vi "Call Check and Download Bitfile.vi"(8 "error in":errorcluster, 9 "Target IP Address":string, 10 "Bitfile Path":path, 11 "Slave Ref":string) -> (0 "error out":errorcluster)   [LabVIEW 2020, in "SEECD System Explorer.lvlib"]
uses:
  SEECD System Explorer.lvlib
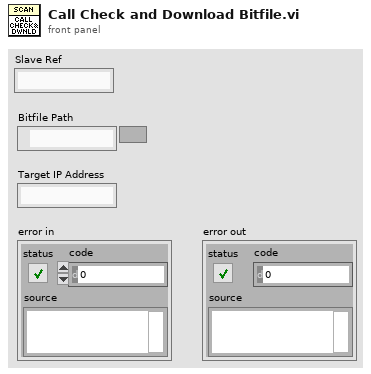
[diagram p1: front panel]
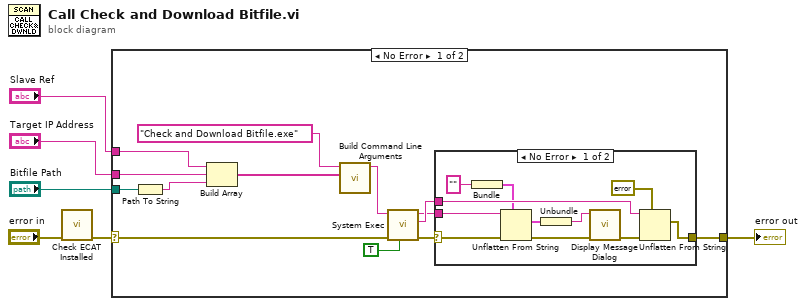
[diagram p0: block diagram]
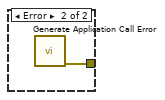
[diagram p2: hidden frame]
diagram:
  n1 = call "Check ECAT Installed.vi"("error in (no error)"="error in") -> ("error out"=w1:errorcluster)  [unwired: 10 in]
  n2 = case shown="No Error" w1 {
    selector: w1 -> [w19 w32]
    tunnel: [w9 w32] -> w2
    tunnel: "Slave Ref" -> [w16 _]
    tunnel: "Target IP Address" -> [w15 _]
    tunnel: "Bitfile Path" -> [w17 _]
    frame No Error {
      n3 = Path To String(path=w17) -> (string=w14:string)
      n4 = Build Array(w16, w15, w14) -> (w13:string[])
      n5 = call "Build Command Line Arguments.vi"("Arguments"=w13, "Executable File Name"="Check and Download Bitfile.exe" ("name or relative path")) -> ("Command Line"=w11:string)  [unwired: 9 in]
      n6 = call <vilib>:"System Exec.vi"("run minimized? (F)"=TRUE, "error in (no error)"=w19, "command line"=w11) -> ("error out"=w10:errorcluster, "standard error"=w8:string, "standard output"=w7:string)  [unwired: 5 in, 1 out]
      n7 = case shown="No Error" w10 {
        selector: w10 -> [w26 _]
        tunnel: [w29 w31] -> w9
        tunnel: w8 -> [w28 _]
        tunnel: w7 -> [w23 _]
        frame No Error {
          n8 = Bundle("") -> (w24:cluster{string})  [unwired: 1 in]
          n9 = Unflatten From String(type=w24, binary string=w23, error in (no error)=w26) -> (value=w21:cluster{string}, error out=w25:errorcluster)  [unwired: 2 in, 1 out]
          n10 = Unbundle(w21) -> (w20:string)
          n11 = call "Display Message Dialog.vi"("error in"=w25, "Message to display"=w20) -> ("error out"=w27:errorcluster)  [unwired: 9 in]
          n12 = Unflatten From String(type=errorcluster {"status"=FALSE, "code"=0, "source"=""} ("error in (no error)"), binary string=w28, error in (no error)=w27) -> (value=w29:errorcluster)  [unwired: 2 in, 2 out]
        }
        frame Error {
          n13 = call "Generate Application Call Error.vi"() -> ("error out"=w31:errorcluster)  [unwired: 11 in]
        }
      }
    }
    frame Error {
    }
  }
  "error out" <- w2
